vi "Suite.vi"(8 "error in (no error)":errorcluster, 10 "LUnit Test Suite in":refnum<class "LUnit Test Suite.lvclass">, 11 "LUnit Test Case In":refnum<class "LUnit Test Case.lvclass">) -> (0 "error out":errorcluster, 2 "LUnit Test Suite Out":refnum<class "LUnit Test Suite.lvclass">, 3 "LUnit Test Case Out":refnum<class "LUnit Test Case.lvclass">)   [LabVIEW 2020, in "LUnit Test Case.lvclass"]
doc: "Factory method to generate a Test Suite object for the test case class.\nThe Test Suite input is used as a collecting parameter to which the test case methods are appended. This can be useful when using custom test suite classes."
uses:
  LUnit Test Case.lvclass
  C:/git/astemes-lunit/source/Runnable.lvclass
  LUnit Test Suite.lvclass
  LUnit Test Case.lvclass/LUnit Test Case.ctl
  C:/git/astemes-lunit/source/LUnit Test Case.lvclass
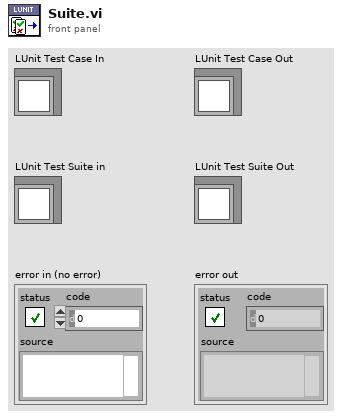
[diagram p1: front panel]
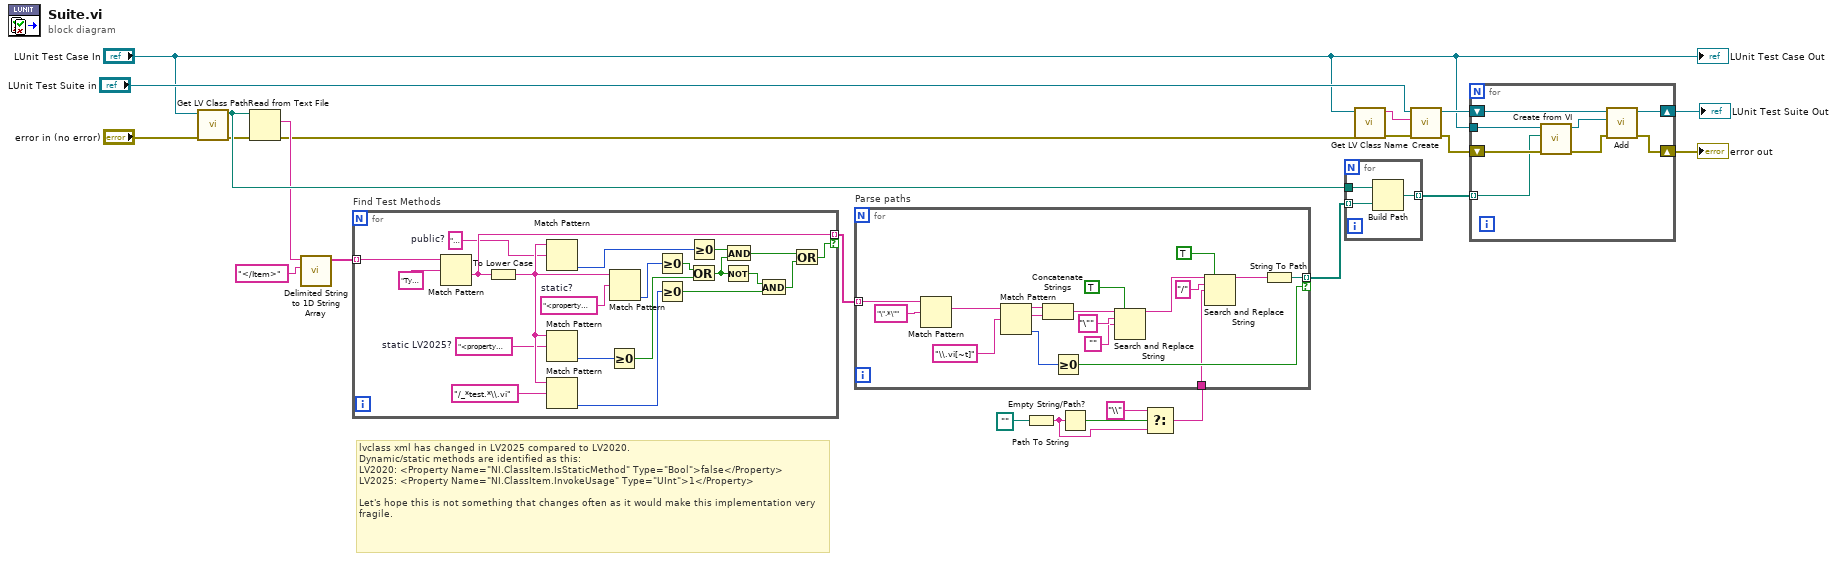
[diagram p0: block diagram]
diagram:
  # "lvclass xml has changed in LV2025 compared to LV2020.\nDynamic/static methods are identified as this:\nLV2020: <Property Name=\"NI.ClassItem.IsStaticMethod\" Type=\"Bool\">false</Property>\nLV2025: <Property Name=\"NI.ClassItem.InvokeUsage\" Type=\"UInt\">1</Property>\n\nLet's hope this is not something that changes often as it would make this implementation very fragile."
  n1 = call <vilib>:"Get LV Class Path.vi"("error in (no error)"="error in (no error)", "object"="LUnit Test Case In") -> ("error out"=w7:errorcluster, "class path"=w14:path)  [unwired: 8 in]
  n2 = Read from Text File(file (use dialog)=w14, error in=w7) -> (text=w8:string, error out=w6:errorcluster)  [unwired: 2 in, 2 out]
  n3 = call <vilib>:"Delimited String to 1D String Array.vi"("delimiter"="</Item>" ("regular expression"), "delimited string"=w8) -> ("string array"=w12:string[])  [unwired: 9 in]
  n4 = for "Find Test Methods" {
    tunnel: w12 -> [w44] mode=indexing
    tunnel: [w40] -> w11 mode=indexing if=w33
    w24 = "<property name=\"ni.classitem.methodscope\" type=\"uint\">1"  # public?
    w28 = "<property name=\"ni.classitem.invokeusage\" type=\"uint\">0"  # static LV2025?
    w43 = "<property name=\"ni.classitem.isstaticmethod\" type=\"bool\">true"  # static?
    n5 = Match Pattern(string=w44, regular expression="Type=\"VI\"") -> (after substring=w40:string)  [unwired: 1 in, 3 out]
    n6 = To Lower Case(string=w40) -> (all lower case string=w29:string)
    n7 = Match Pattern(string=w29, regular expression=w24) -> (offset past match=w41:i32)  [unwired: 1 in, 3 out]
    n8 = Match Pattern(string=w29, regular expression=w28) -> (offset past match=w30:i32)  [unwired: 1 in, 3 out]
    n9 = Match Pattern(string=w29, regular expression="/_*test.*\\.vi") -> (offset past match=w37:i32)  [unwired: 1 in, 3 out]
    n10 = Greater Or Equal To 0?(x=w30) -> (x >= 0?=w26:bool)
    n11 = Match Pattern(string=w29, regular expression=w43) -> (offset past match=w42:i32)  [unwired: 1 in, 3 out]
    n12 = Greater Or Equal To 0?(x=w42) -> (x >= 0?=w36:bool)
    n13 = Greater Or Equal To 0?(x=w37) -> (x >= 0?=w34:bool)
    n14 = Greater Or Equal To 0?(x=w41) -> (x >= 0?=w39:bool)
    n15 = Or(x=w36, y=w26) -> (x .or. y?=w27:bool)
    n16 = Not(x=w27) -> (.not. x?=w35:bool)
    n17 = And(x=w39, y=w27) -> (x .and. y?=w32:bool)
    n18 = And(x=w35, y=w34) -> (x .and. y?=w31:bool)
    n19 = Or(x=w32, y=w31) -> (x .or. y?=w33:bool)
  }
  n20 = Path To String(path=path "") -> (string=w1:string)
  n21 = Empty String/Path?(string/path=w1) -> (empty?=w3:bool)
  n22 = Select(t="\\" ("search string"), s=w3, f=w1) -> (s? t:f=w5:string)
  n23 = for "Parse paths" {
    tunnel: w11 -> [w62] mode=indexing
    tunnel: [w57] -> w9 mode=indexing if=w48
    tunnel: w5 -> [w45]
    n24 = Match Pattern(string=w62, regular expression="\".*\"") -> (match substring=w51:string)  [unwired: 1 in, 3 out]
    n25 = Match Pattern(string=w51, regular expression="\\.vi[~t]") -> (before substring=w53:string, match substring=w52:string, offset past match=w49:i32)  [unwired: 1 in, 1 out]
    n26 = Concatenate Strings(w53, w52) -> (w50:string)
    n27 = Greater Or Equal To 0?(x=w49) -> (x >= 0?=w48:bool)
    n28 = Search and Replace String(replace all?=TRUE ("replace all? (F)"), input string=w50, search string="\"", replace string="") -> (result string=w56:string)  [unwired: 4 in, 3 out]
    n29 = Search and Replace String(replace all?=TRUE ("replace all? (F)"), input string=w56, search string="/", replace string=w45) -> (result string=w55:string)  [unwired: 4 in, 3 out]
    n30 = String To Path(string=w55) -> (path=w57:path)
  }
  n31 = for {
    tunnel: w14 -> [w65]
    tunnel: w9 -> [w64] mode=indexing
    tunnel: [w63] -> w13 mode=indexing
    n32 = Build Path(base path=w65, name or relative path=w64) -> (appended path=w63:path)
  }
  n33 = call <vilib>:"Get LV Class Name.vi"("error in (no error)"=w6, "object"="LUnit Test Case In") -> ("error out"=w15:errorcluster, "class name"=w16:string)  [unwired: 8 in]
  n34 = call "Create.vi"("error in (no error)"=w15, "Suite Name"=w16, "LUnit Test Suite in"="LUnit Test Suite in") -> ("error out"=w22:errorcluster, "LUnit Test Suite Out"=w23:refnum<class "LUnit Test Suite.lvclass">)  [unwired: 7 in]
  n35 = for {
    tunnel: w13 -> [w66] mode=indexing
    shift-right: [w72] -> w21
    shift-left: w23 -> [w73]
    shift-right: [w70] -> w19
    shift-left: w22 -> [w69]
    tunnel: "LUnit Test Case In" -> [w67]
    n36 = call "Create from VI.vi"("error in (no error)"=w69, "Test Method VI Path"=w66, "LUnit Test Case In"=w67) -> ("error out"=w71:errorcluster, "LUnit Test Case Out"=w68:refnum<class "LUnit Test Case.lvclass">)  [unwired: 7 in]
    n37 = call "Add.vi"("error in (no error)"=w71, "Runnable"=w68, "LUnit Test Suite In"=w73) -> ("error out"=w70:errorcluster, "LUnit Test Suite Out"=w72:refnum<class "LUnit Test Suite.lvclass">)  [unwired: 7 in]
  }
  "error out" <- w19
  "LUnit Test Suite Out" <- w21
  "LUnit Test Case Out" <- "LUnit Test Case In"
